vi "DialogCloneClass.vi"(0 "ClassWriterNative.lvclass":refnum<class "ClassWriterNative.lvclass">, 1 "ClassItemRefIn":refnum<vi>, 5 "error in (no error)":errorcluster) -> (14 "ClassWriterGOOP300.lvclassOut":refnum<class "ClassWriterNative.lvclass">, 15 "ClassItemRefOut":refnum<vi>, 16 "NewClassPath":path, 17 "Cancelled":bool, 19 "error out":errorcluster)   [LabVIEW 2020, in "ClassWriterNative.lvclass"]
uses:
  ClassWriterNative.lvclass
  ed2075f3-ccba-4581-8a34-503f5f924372.vi
  <vilib>/Utility/lvfile.llb/NI_FileType.lvlib
panel:
  in  "Help":bool
  out "ProductPicture":picture
  in  "_ShowContextHelp":bool
  in  "_UseClassSuffix":string caption="Class Folder Suffix"
  in  "_NewClassPath":path caption="New Class Folder"
  in  "_NewClassName":string caption="New Class Name"
  out "_DubName":string caption="This name already exists"
  in  "_Cancel":bool
  in  "_CloneClass":bool
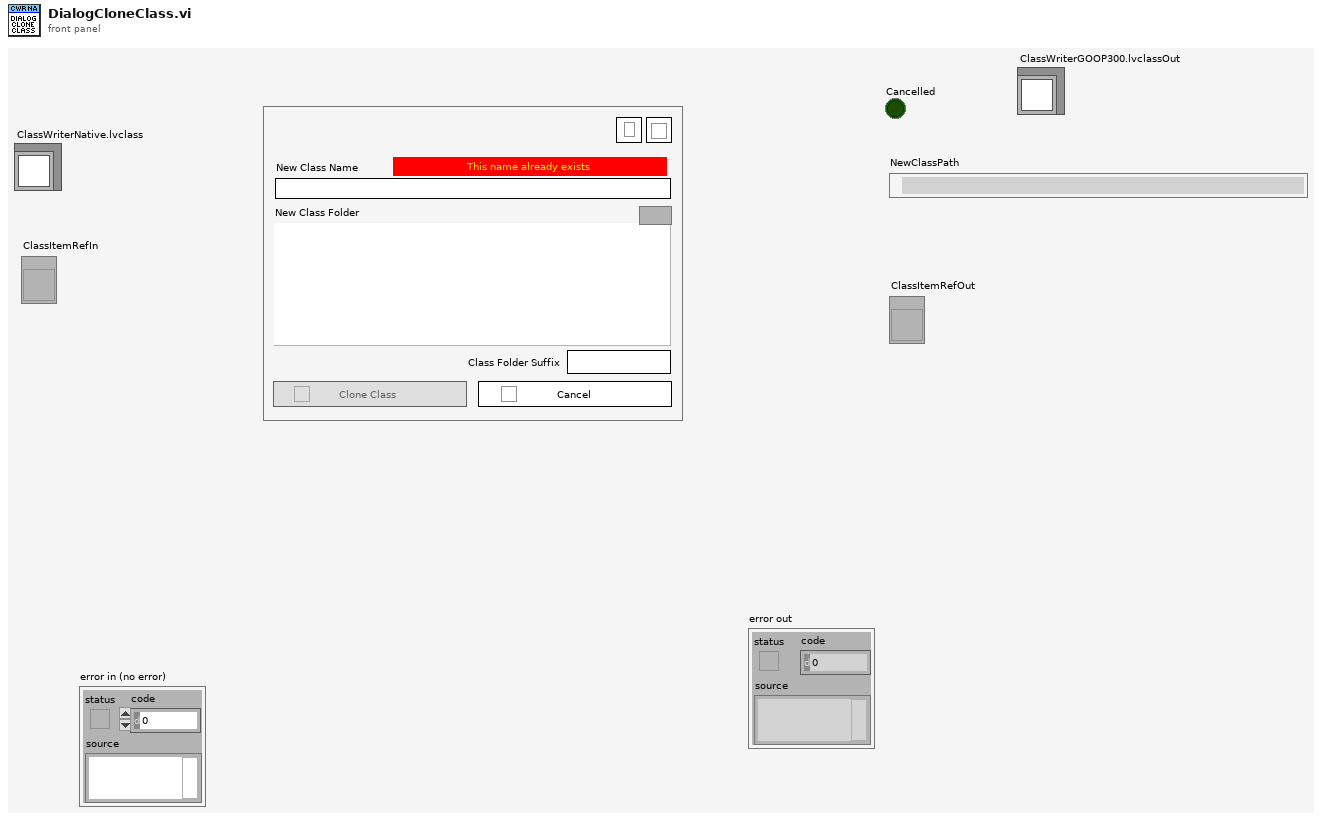
[diagram p1: front panel]
types:
  T1 = cluster{"Cancel":bool, "OrgClassPath":path, "ClassName":string, "Interface":bool}
  T2 = typedef "BaseProvider_IniFileSettings.ctl" = cluster{"ClassFolderSuffix":string, "InterfaceFolderSuffix":string, "InterfaceIcon":string, "FileNamingOption":T3, "DynamicDispatchStartValue":bool}
  T3 = typedef "BaseProvider_FileNamingOption.ctl" = enum16{"CamelCase", "Space", "Underscore"}
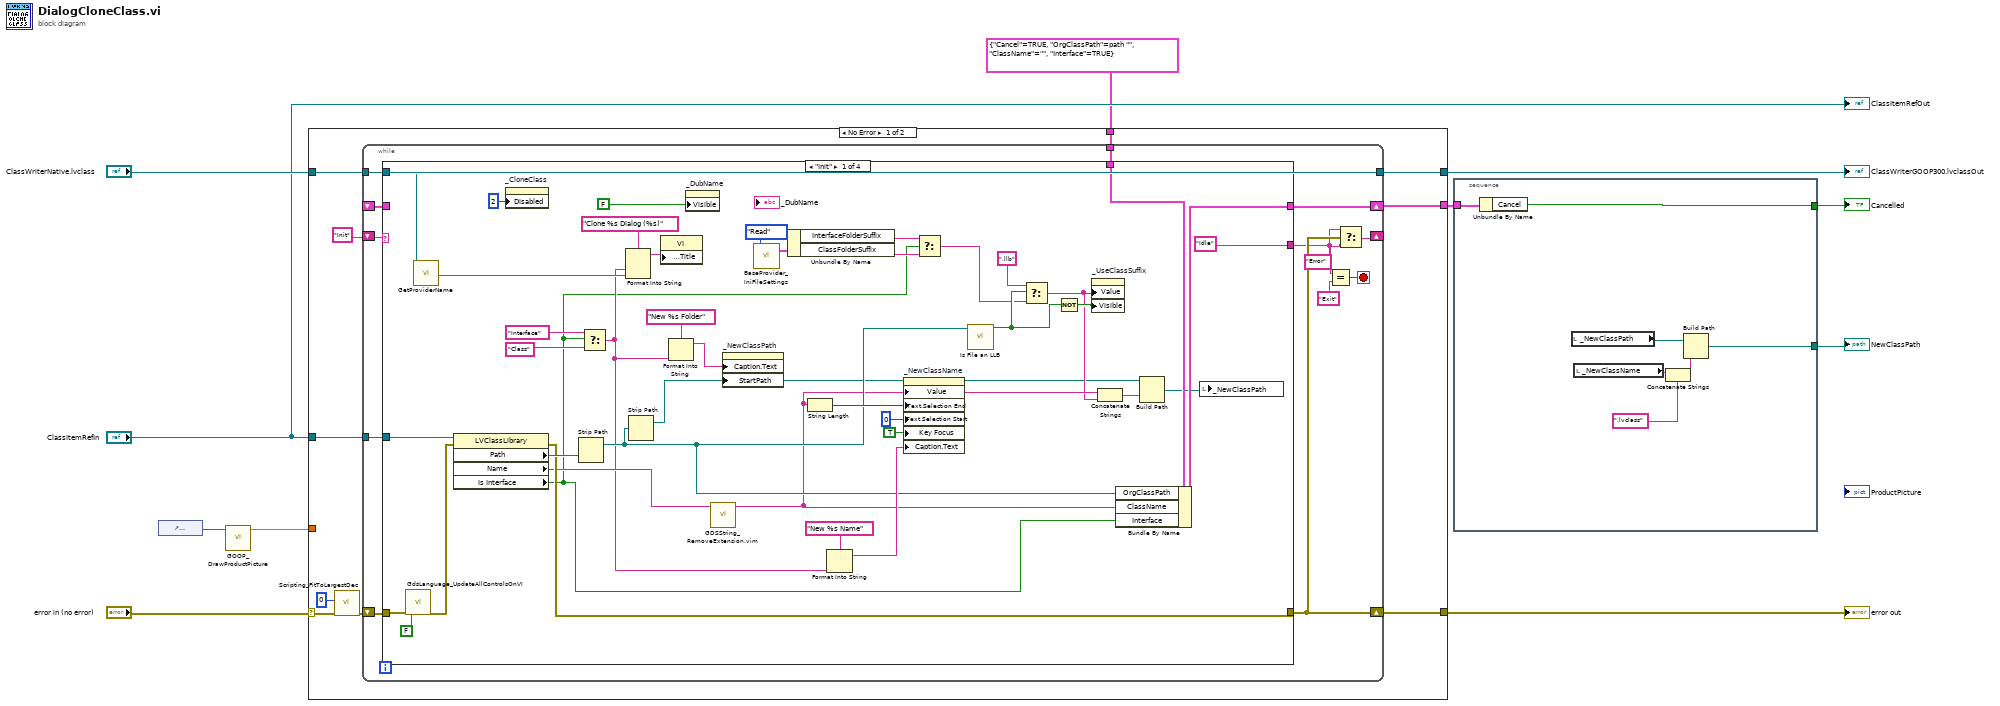
[diagram p0: block diagram]
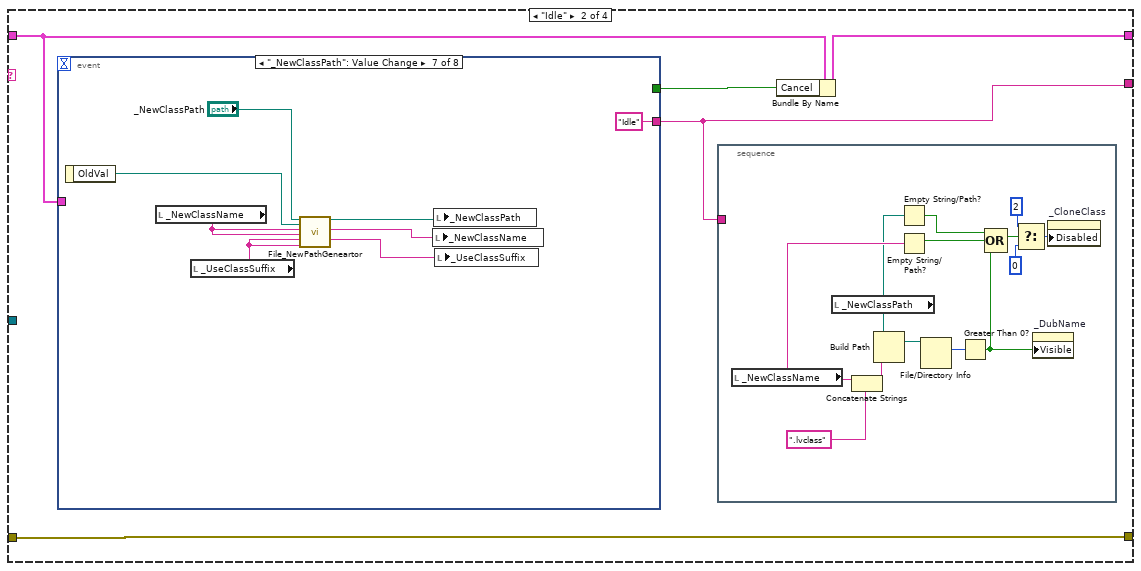
[diagram p2: hidden frame]
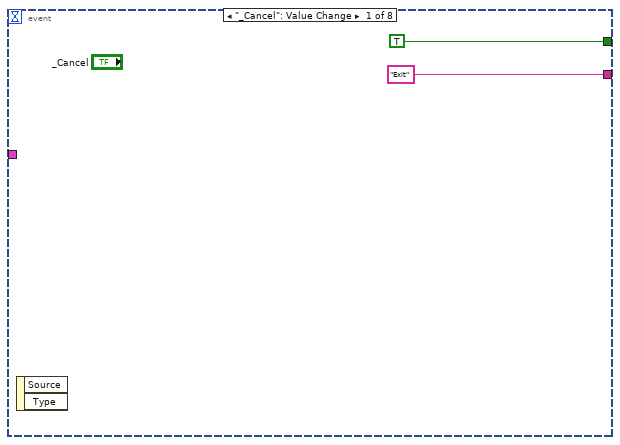
[diagram p3: hidden frame]
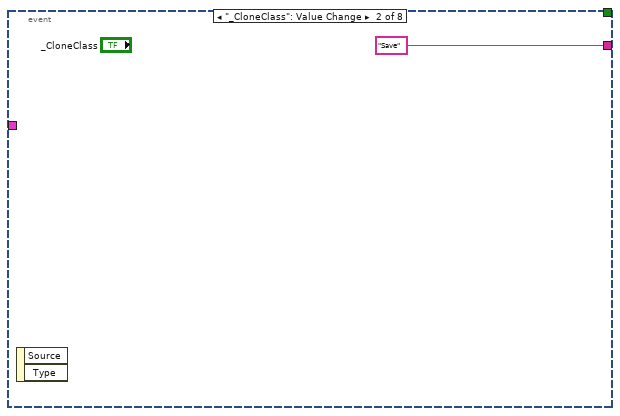
[diagram p4: hidden frame]
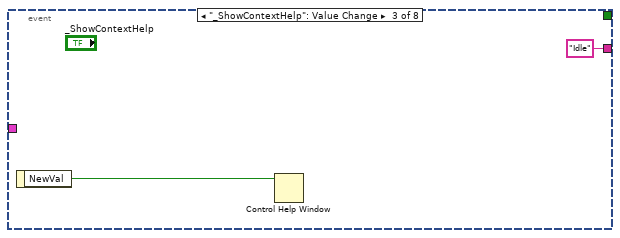
[diagram p5: hidden frame]
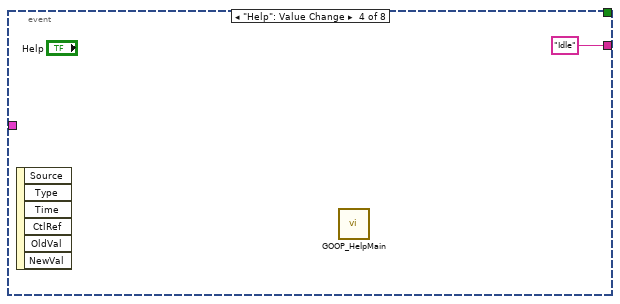
[diagram p6: hidden frame]
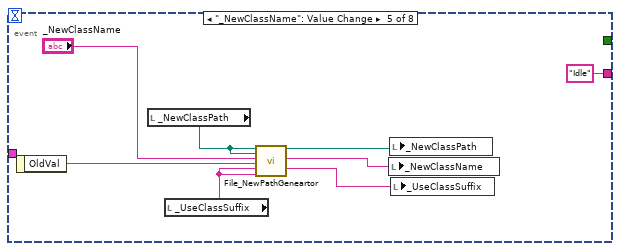
[diagram p7: hidden frame]
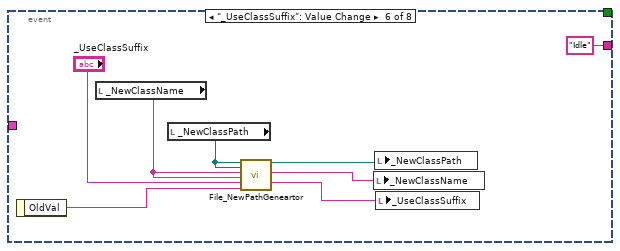
[diagram p8: hidden frame]
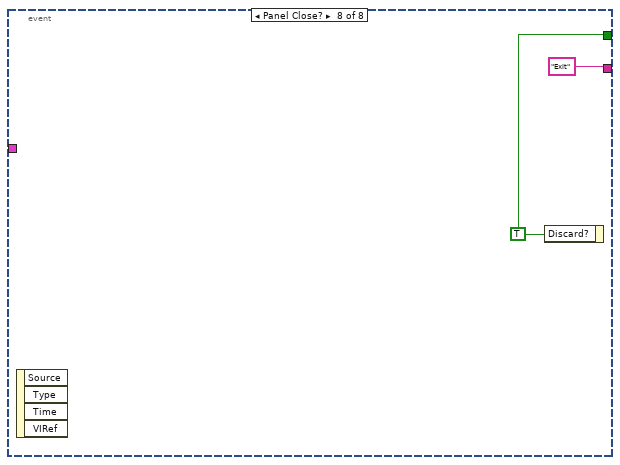
[diagram p9: hidden frame]
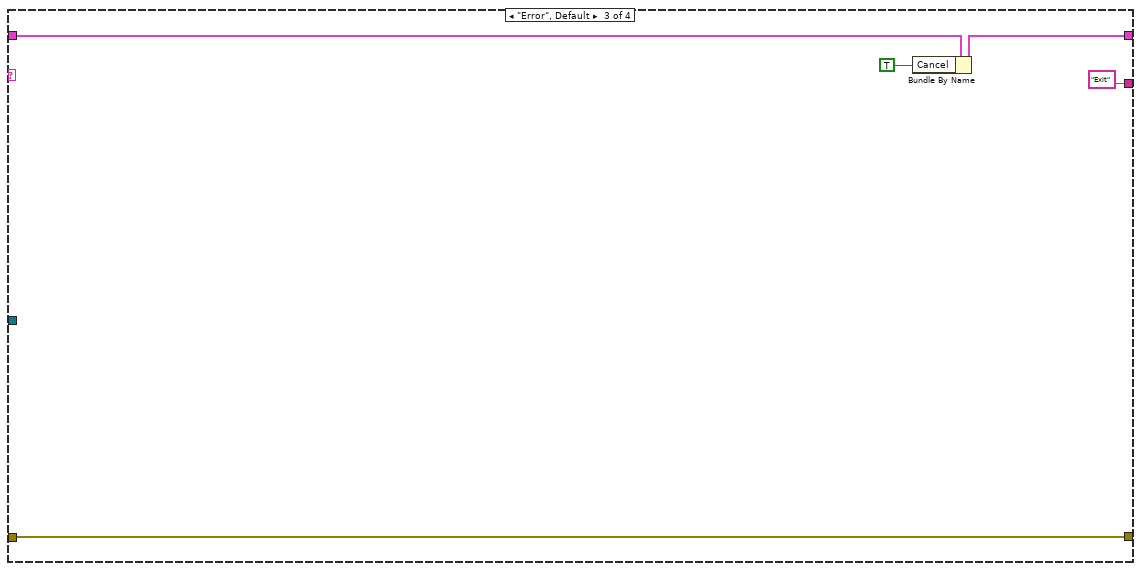
[diagram p10: hidden frame]
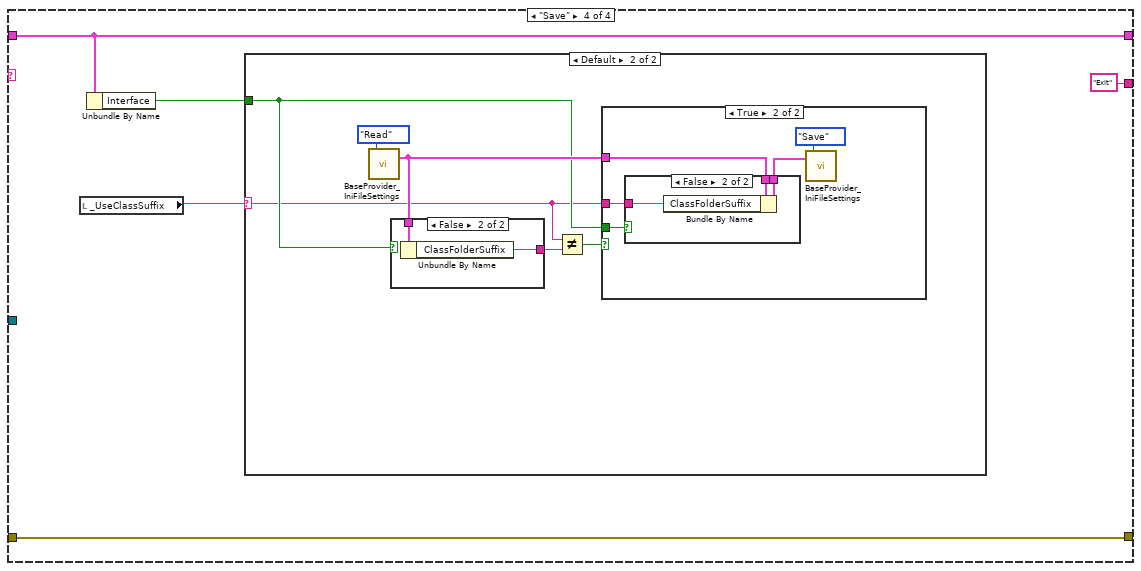
[diagram p11: hidden frame]
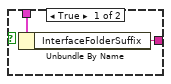
[diagram p13: hidden frame]
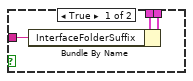
[diagram p15: hidden frame]
diagram:
  n1 = control-ref of="ProductPicture"() -> (w2:refnum<vi>)
  n2 = call "GOOP_DrawProductPicture.vi"("ProductPictureControl"=w2) -> ("Zoom Factor"=w1:sgl)  [unwired: 10 in]
  n3 = case shown="No Error" "error in (no error)" {
    selector: "error in (no error)" -> [w13 w158]
    tunnel: "ClassWriterNative.lvclass" -> [w18 w157]
    tunnel: [w21 w158] -> w5
    tunnel: [w19 w157] -> w9
    tunnel: T1 {"Cancel"=TRUE, "OrgClassPath"=path "", "ClassName"="", "Interface"=TRUE} ("output cluster") -> [w17 _]
    tunnel: "ClassItemRefIn" -> [w16 _]
    tunnel: [w15 _] -> w8
    tunnel: w1 -> [_ _]
    frame No Error {
      n4 = call "Scripting_FitToLargestDec.vi"("error in (no error)"=w13, "border spacing (2 px)"=0) -> ("error out"=w12:errorcluster)  [unwired: 4 in, 1 out]
      n5 = while {
        shift-right: [w28] -> w21
        shift-left: w12 -> [w34]
        shift-right: [w27] -> _
        shift-left: "Init" -> [w31]
        shift-right: [w32] -> w15
        shift-left: _ -> [w33]
        tunnel: w18 -> [w24]
        tunnel: [w24] -> w19
        tunnel: w17 -> [w23]
        tunnel: w16 -> [w22]
        stop <- w29 stop-if-true
        n6 = case shown="\"Init\"" w31 {
          tunnel: w33 -> [_ w76 w128 w133]
          tunnel: [w74 w78 w127 w133] -> w32
          tunnel: w34 -> [w62 w80 w129 w134]
          tunnel: [w68 w80 w129 w134] -> w28
          tunnel: w24 -> [w63 _ _ _]
          tunnel: ["Idle" w79 "Exit" "Exit"] -> w26
          tunnel: w23 -> [w72 _ _ _]
          tunnel: w22 -> [w73 _ _ _]
          frame "Init" {
            n7 = call "GdsLanguage_UpdateAllControlsOnVI.vi"("error in (no error)"=w62, "CreateLanguageFile(Use this to create a languageFile)"=FALSE) -> ("error out"=w61:errorcluster)  [unwired: 16 in, 1 out]
            n8 = call-dynamic "GetProviderName.vi"("ClassWriterNative in"=w63) -> ("TranslatedProviderName"=w56:string)  [unwired: 15 in, 3 out]
            n9 = property class="LVClassLibrary"(reference=w73, error in=w61) -> (error out=w68:errorcluster, "Path"=w70:path, "Name"=w52:string, "Is Interface"=w41:bool)  [unwired: 1 out]
            n10 = property on="_CloneClass" class="Bool"("Disabled"=u8 2) -> ()  [unwired: 2 in, 2 out]
            n11 = Strip Path(path=w70) -> (stripped path=w49:path)  [unwired: 1 out]
            n12 = Select(t="Interface", s=w41, f="Class") -> (s? t:f=w48:string)
            n13 = Format Into String(format string="Clone %s Dialog (%s)", w48, w56) -> (resulting string=w64:string)  [unwired: 2 in, 1 out]
            n14 = Strip Path(path=w49) -> (stripped path=w37:path)  [unwired: 1 out]
            n15 = property class="VI"("Front Panel.Title"=w64) -> ()  [unwired: 2 in, 2 out]
            n16 = Format Into String(format string="New %s Folder", w48) -> (resulting string=w46:string)  [unwired: 2 in, 1 out]
            n17 = property on="_DubName" class="Str"("Visible"=FALSE) -> ()  [unwired: 2 in, 2 out]
            n18 = call "GDSString_RemoveExtension.vim"("NameWithExtension"=w52) -> ("NameWithoutExtension"=w39:string)  [unwired: 9 in, 1 out]
            n19 = property on="_NewClassPath" class="Path"("Caption.Text"=w46, "StartPath"=w37) -> ()  [unwired: 2 in, 2 out]
            n20 = call "BaseProvider_IniFileSettings.vi"("Action"=enum16{"Read", "Load", "Save"}."Read") -> ("IniFileSettings"=w44:T2)  [unwired: 17 in, 1 out]
            n21 = Unbundle By Name(w44) -> ("InterfaceFolderSuffix"=w43:string, "ClassFolderSuffix"=w42:string)
            n22 = String Length(string=w39) -> (length=w65:i32)
            n23 = Format Into String(format string="New %s Name", w48) -> (resulting string=w50:string)  [unwired: 2 in, 1 out]
            n24 = property on="_NewClassName" class="Str"("Value"=w39, "Text.Selection End"=w65, "Text.Selection Start"=u32 0 ("Text.Selection:Start"), "Key Focus"=TRUE, "Caption.Text"=w50) -> ()  [unwired: 2 in, 2 out]
            n25 = Select(t=w43, s=w41, f=w42) -> (s? t:f=w40:string)
            n26 = call <vilib>:"Is File an LLB.vi"("path"=w49) -> ("Is LLB?"=w57:bool)  [unwired: 9 in, 1 out]
            n27 = Select(t=".llb" ("y"), s=w57, f=w40) -> (s? t:f=w38:string)
            n28 = Not(x=w57) -> (.not. x?=w59:bool)
            n29 = property on="_UseClassSuffix" class="Str"("Value"=w38, "Visible"=w59) -> ()  [unwired: 2 in, 2 out]
            n30 = Concatenate Strings(w39, w38) -> (w36:string)
            n31 = Bundle By Name(cluster=w72, "OrgClassPath"=w49, "ClassName"=w39, "Interface"=w41) -> (w74:T1)
            n32 = Build Path(base path=w37, name or relative path=w36) -> (appended path=w35:path)
            n33 = local write "_NewClassPath"(w35) -> ()
          }
          frame "Idle" {
            n34 = event shown="[6] \"_NewClassPath\": Value Change" {
              selector: _ -> [_ _ _ _ _ _ _ _]
              dyn-events: _ -> [_ _ _ _ _ _ _ _]
              timeout: _ -> [_ _ _ _ _ _ _ _]
              tunnel: ["Exit" "Save" "Idle" "Idle" "Idle" "Idle" "Idle" "Exit"] -> w79
              tunnel: [TRUE _ _ _ _ _ _ w125] -> w77
              tunnel: w76 -> [_ _ _ _ _ _ _ _]
              event "_Cancel": Value Change {
                n35 = event-data() -> ()  [unwired: 1 in, 2 out]
              }
              event "_CloneClass": Value Change {
                n36 = event-data() -> ()  [unwired: 1 in, 2 out]
              }
              event "_ShowContextHelp": Value Change {
                n37 = event-data() -> ("NewVal"=w97:bool)  [unwired: 1 in]
                n38 = Control Help Window(1:w97) -> ()  [unwired: 1 in]
              }
              event "Help": Value Change {
                n39 = event-data() -> ()  [unwired: 1 in, 6 out]
                n40 = call "GOOP_HelpMain.vi"() -> ()  [unwired: 12 in]
              }
              event "_NewClassName": Value Change {
                n41 = event-data() -> ("OldVal"=w103:string)  [unwired: 1 in]
                n42 = local read "_NewClassPath"() -> (w106:path)
                n43 = local read "_UseClassSuffix"() -> (w102:string)
                n44 = call "File_NewPathGeneartor.vi"("NewPath"=w106, "OldPath"=w106, "NewName"="_NewClassName", "OldName"=w103, "NewSuffix"=w102, "OldSuffix"=w102) -> ("PathOut"=w105:path, "NameOut"=w101:string, "SuffixOut"=w100:string)  [unwired: 11 in]
                n45 = local write "_NewClassName"(w101) -> ()
                n46 = local write "_NewClassPath"(w105) -> ()
                n47 = local write "_UseClassSuffix"(w100) -> ()
              }
              event "_UseClassSuffix": Value Change {
                n48 = event-data() -> ("OldVal"=w108:string)  [unwired: 1 in]
                n49 = local read "_NewClassName"() -> (w110:string)
                n50 = local read "_NewClassPath"() -> (w111:path)
                n51 = call "File_NewPathGeneartor.vi"("NewPath"=w111, "OldPath"=w111, "NewName"=w110, "OldName"=w110, "NewSuffix"="_UseClassSuffix", "OldSuffix"=w108) -> ("PathOut"=w114:path, "NameOut"=w113:string, "SuffixOut"=w112:string)  [unwired: 11 in]
                n52 = local write "_NewClassName"(w113) -> ()
                n53 = local write "_NewClassPath"(w114) -> ()
                n54 = local write "_UseClassSuffix"(w112) -> ()
              }
              event "_NewClassPath": Value Change {
                n55 = event-data() -> ("OldVal"=w117:path)  [unwired: 1 in]
                n56 = local read "_NewClassName"() -> (w119:string)
                n57 = local read "_UseClassSuffix"() -> (w116:string)
                n58 = call "File_NewPathGeneartor.vi"("NewPath"="_NewClassPath", "OldPath"=w117, "NewName"=w119, "OldName"=w119, "NewSuffix"=w116, "OldSuffix"=w116) -> ("PathOut"=w122:path, "NameOut"=w121:string, "SuffixOut"=w120:string)  [unwired: 11 in]
                n59 = local write "_NewClassName"(w121) -> ()
                n60 = local write "_NewClassPath"(w122) -> ()
                n61 = local write "_UseClassSuffix"(w120) -> ()
              }
              event Panel Close? {
                w125 = TRUE ("Discard?")
                n62 = event-data() -> ()  [unwired: 1 in, 4 out]
                n63 = event-data("Discard?"=w125) -> ()  [unwired: 1 in, 1 out]
              }
            }
            n64 = stacked-sequence {
              tunnel: w79 -> [_]
              frame #0 {
                n65 = local read "_NewClassName"() -> (w84:string)
                n66 = local read "_NewClassPath"() -> (w82:path)
                n67 = Concatenate Strings(w84, ".lvclass" ("string")) -> (w88:string)
                n68 = Build Path(base path=w82, name or relative path=w88) -> (appended path=w87:path)
                n69 = Empty String/Path?(string/path=w82) -> (empty?=w81:bool)
                n70 = Empty String/Path?(string/path=w84) -> (empty?=w83:bool)
                n71 = File/Directory Info(path=w87) -> (size=w86:i64)  [unwired: 1 in, 6 out]
                n72 = Greater Than 0?(x=w86) -> (x > 0?=w85:bool)
                n73 = Compound Arithmetic op=OR(w81, w83, w85) -> (w90:bool)
                n74 = Select(t=u8 2, s=w90, f=u8 0 ("Disabled")) -> (s? t:f=w93:u8)
                n75 = property on="_DubName" class="Str"("Visible"=w85) -> ()  [unwired: 2 in, 2 out]
                n76 = property on="_CloneClass" class="Bool"("Disabled"=w93) -> ()  [unwired: 2 in, 2 out]
              }
            }
            n77 = Bundle By Name(cluster=w76, "Cancel"=w77) -> (w78:T1)
          }
          frame "Error", Default {
            n78 = Bundle By Name(cluster=w128, "Cancel"=TRUE) -> (w127:T1)
          }
          frame "Save" {
            n79 = local read "_UseClassSuffix"() -> (w131:string)
            n80 = Unbundle By Name(w133) -> ("Interface"=w132:bool)
            n81 = case shown="Default" w131 {
              selector: w131 -> [_ w136]
              tunnel: w132 -> [_ w137]
              frame ".llb" {
              }
              frame Default {
                n82 = call "BaseProvider_IniFileSettings.vi"("Action"=enum16{"Read", "Load", "Save"}."Read") -> ("IniFileSettings"=w140:T2)  [unwired: 17 in, 1 out]
                n83 = case shown="False" w137 {
                  tunnel: [w143 w145] -> w139
                  tunnel: w140 -> [w142 w144]
                  frame True {
                    n84 = Unbundle By Name(w142) -> ("InterfaceFolderSuffix"=w143:string)
                  }
                  frame False {
                    n85 = Unbundle By Name(w144) -> ("ClassFolderSuffix"=w145:string)
                  }
                }
                n86 = Not Equal?(x=w136, y=w139) -> (x != y?=w141:bool)
                n87 = case shown="True" w141 {
                  tunnel: w140 -> [_ w148]
                  tunnel: w136 -> [_ w147]
                  tunnel: w137 -> [_ w146]
                  frame False {
                  }
                  frame True {
                    n88 = case shown="False" w146 {
                      tunnel: [w153 w156] -> w150
                      tunnel: w148 -> [w152 w155]
                      tunnel: w147 -> [w151 w154]
                      frame True {
                        n89 = Bundle By Name(cluster=w152, "InterfaceFolderSuffix"=w151) -> (w153:T2)
                      }
                      frame False {
                        n90 = Bundle By Name(cluster=w155, "ClassFolderSuffix"=w154) -> (w156:T2)
                      }
                    }
                    n91 = call "BaseProvider_IniFileSettings.vi"("IniFileSettings"=w150, "Action"=enum16{"Read", "Load", "Save"}."Save") -> ()  [unwired: 16 in, 2 out]
                  }
                }
              }
            }
          }
        }
        n92 = Equal?(x=w26, y="Exit") -> (x = y?=w29:bool)
        n93 = Select(t="Error", s=w28, f=w26) -> (s? t:f=w27:string)
      }
    }
    frame Error {
    }
  }
  "ClassWriterGOOP300.lvclassOut" <- w9
  "error out" <- w5
  n94 = stacked-sequence {
    tunnel: w8 -> [w164]
    tunnel: [w165] -> w7
    tunnel: [w159] -> w3
    frame #0 {
      n95 = Unbundle By Name(w164) -> ("Cancel"=w165:bool)
      n96 = local read "_NewClassPath"() -> (w163:path)
      n97 = local read "_NewClassName"() -> (w162:string)
      n98 = Concatenate Strings(w162, ".lvclass" ("string")) -> (w161:string)
      n99 = Build Path(base path=w163, name or relative path=w161) -> (appended path=w159:path)
    }
  }
  "Cancelled" <- w7
  "NewClassPath" <- w3
  "ClassItemRefOut" <- "ClassItemRefIn"
